vi "GOOP_AddCustomClassTemplates.vi"(7 "DerivedFromThisClass(if any)":refnum<vi>, 9 "BuildInTemplates":string[](array[string]), 10 "TemplateIdNamesIn":T2[](array[typedef]), 11 "ClassWriter in":refnum<class "ClassWriter.lvclass">) -> (2 "TemplateIdNamesOut":T2[](array[typedef]))   [LabVIEW 2020]
uses:
  <resource>/Framework/Providers/Open_GDS/ClassProviders/Provider_BaseClassInterface/ClassTemplateType.ctl
  <resource>/Framework/Providers/Open_GDS/ClassProviders/Provider_BaseClassInterface/ClassWriter_class/ClassWriter.lvclass
  <resource>/Framework/Providers/Open_GDS/ClassProviders/Common/ScriptingFunctions/Scripting_ConnectorPanePatternType.ctl
panel:
  out "PatternOut":T1 items=["4x4x4", "5x6x5", "6x8x6"]
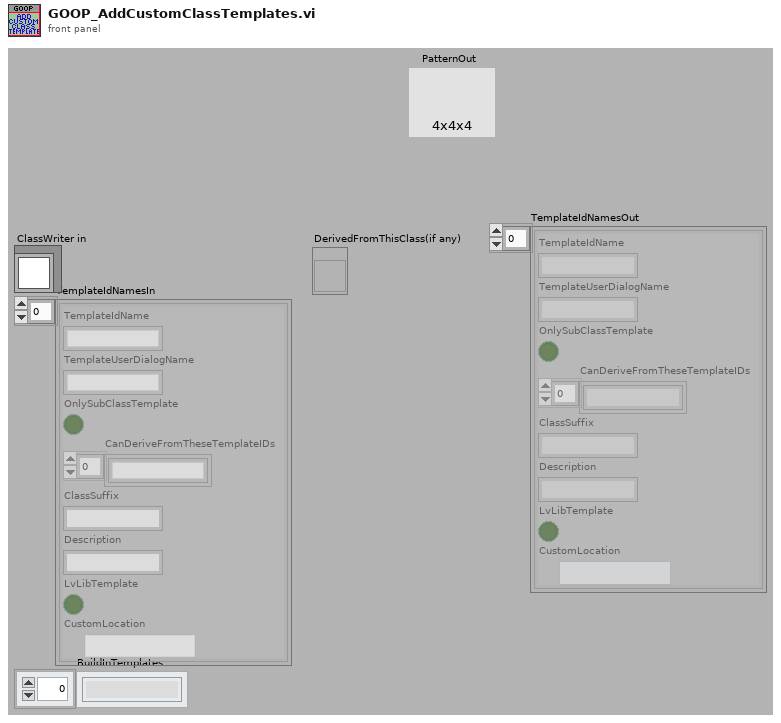
[diagram p1: front panel]
types:
  T1 = typedef "Scripting_ConnectorPanePatternType.ctl" = u16
  T2 = typedef "ClassWriter.lvclass/ClassTemplateType.ctl" = cluster{"TemplateIdName":string, "TemplateUserDialogName":string, "OnlySubClassTemplate":bool, "CanDeriveFromTheseTemplateIDs":string[], "ClassSuffix":string, "Description":string, "LvLibTemplate":bool, "CustomLocation":path}
  T3 = typedef "GDSLvCLass_ClassSettingsType.ctl" = cluster{"ClassProviderName":string, "ClassTemplateUsed":string, "ClassTemplateVersion":string, "ClassDescription":string, "PlugIns":T4[], "ConnectorPanePattern":string}
  T4 = typedef "GDSLvClass_PlugIn.ctl" = cluster{"Type":T5, "ID":string, "Version":string, "Path":path, "Name":string, "Data":variant}
  T5 = typedef "GDSLvClass_PlugInTypes.ctl" = enum16{"DesignPattern", "MethodTypes"}
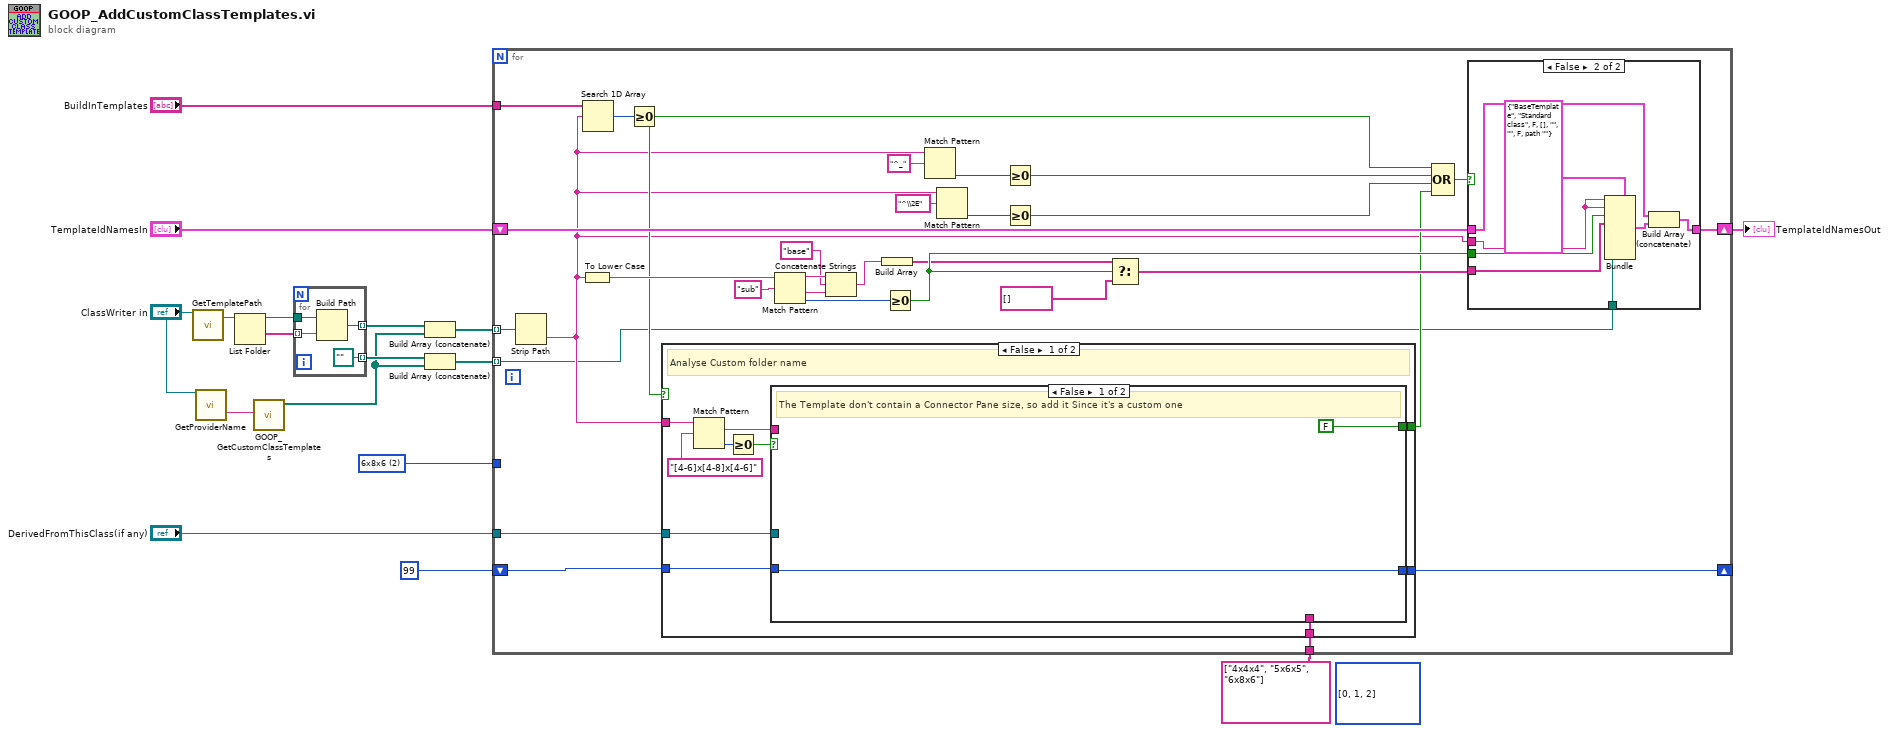
[diagram p0: block diagram]
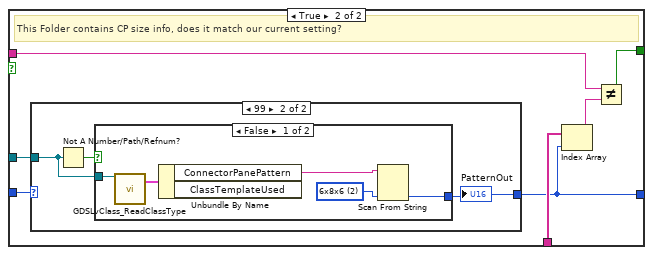
[diagram p2: hidden frame]
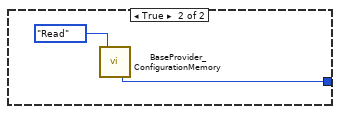
[diagram p4: hidden frame]
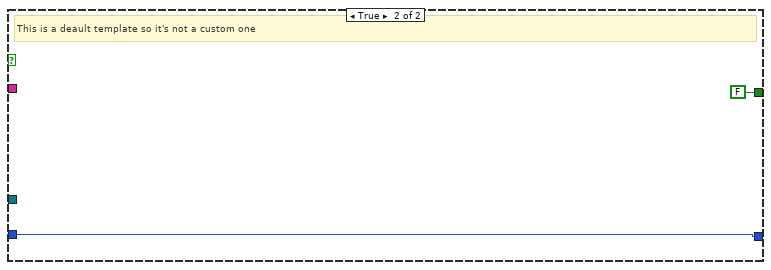
[diagram p5: hidden frame]
diagram:
  w11 = T1 2 items=["4x4x4", "5x6x5", "6x8x6"] ("_DefaultConnectorPanePattern")
  (unwired) T1[] [0, 1, 2] items=["4x4x4", "5x6x5", "6x8x6"] ("Pattern")
  n1 = call-dynamic "GetTemplatePath.vi"("ClassWriterIn"="ClassWriter in") -> ("FolderPathOut"=w15:path)  [unwired: 14 in, 4 out]
  n2 = call-dynamic "GetProviderName.vi"("ClassWriter in"="ClassWriter in") -> ("ShortName(Could be used in for INI Sections)"=w6:string)  [unwired: 14 in, 4 out]
  n3 = List Folder(path=w15) -> (path out=w8:path, folder names=w13:string[])  [unwired: 3 in, 2 out]
  n4 = call <resource>:"GOOP_GetCustomClassTemplates.vi"("ClassType"=w6) -> ("CustomTemplates"=w2:path[])  [unwired: 10 in]
  n5 = for {
    tunnel: w13 -> [w21] mode=indexing
    tunnel: w8 -> [w20]
    tunnel: [w19] -> w4 mode=indexing
    tunnel: [path ""] -> w3 mode=indexing
    n6 = Build Path(base path=w20, name or relative path=w21) -> (appended path=w19:path)
  }
  n7 = Build Array (concatenate)(w4, w2) -> (w5:path[])
  n8 = Build Array (concatenate)(w3, w2) -> (w1:path[])
  n9 = for {
    tunnel: "BuildInTemplates" -> [w32]
    shift-right: [w42] -> w16
    shift-left: "TemplateIdNamesIn" -> [w43]
    shift-right: [w28] -> _
    shift-left: u16 99 -> [w30]
    tunnel: w11 -> [_]
    tunnel: "DerivedFromThisClass(if any)" -> [w29]
    tunnel: string[] ["4x4x4", "5x6x5", "6x8x6"] ("Pattern") -> [w25]
    tunnel: w5 -> [w24] mode=indexing
    tunnel: w1 -> [w22] mode=indexing
    n10 = Strip Path(path=w24) -> (name=w23:string)  [unwired: 1 out]
    n11 = To Lower Case(string=w23) -> (all lower case string=w31:string)
    n12 = Search 1D Array(1D array=w32, element=w23) -> (index of element=w33:i32)  [unwired: 1 in]
    n13 = Greater Or Equal To 0?(x=w33) -> (x >= 0?=w26:bool)
    n14 = case shown="False" w26 {
      tunnel: w23 -> [w62 _]
      tunnel: w30 -> [w58 w84]
      tunnel: w29 -> [w57 _]
      tunnel: [w56 w84] -> w28
      tunnel: [w55 FALSE] -> w27
      tunnel: w25 -> [w54 _]
      frame False {
        # "Analyse Custom folder name"
        n15 = Match Pattern(string=w62, regular expression="[4-6]x[4-8]x[4-6]") -> (match substring=w53:string, offset past match=w60:i32)  [unwired: 1 in, 2 out]
        n16 = Greater Or Equal To 0?(x=w60) -> (x >= 0?=w59:bool)
        n17 = case shown="False" w59 {
          tunnel: w58 -> [w64 w71]
          tunnel: w57 -> [_ w70]
          tunnel: [w64 w68] -> w56
          tunnel: [FALSE w65] -> w55
          tunnel: w54 -> [_ w69]
          tunnel: w53 -> [_ w66]
          frame False {
            # "The Template don't contain a Connector Pane size, so add it Since it's a custom one"
          }
          frame True {
            # "This Folder contains CP size info, does it match our current setting?"
            n18 = case shown="99" w71 {
              selector: w71 -> [w72 _]
              tunnel: w70 -> [_ w74]
              tunnel: [w72 w73] -> w68
              frame 0, Default {
              }
              frame 99 {
                n19 = Not A Number/Path/Refnum?(number/path/refnum=w74) -> (NaN/Path/Refnum?=w75:bool)
                n20 = case shown="False" w75 {
                  tunnel: w74 -> [w77 _]
                  tunnel: [w76 w81] -> w73
                  frame False {
                    w78 = T1 2 items=["4x4x4", "5x6x5", "6x8x6"] ("Pattern")
                    n21 = call <resource>:"GDSLvClass_ReadClassType.vi"("Class Refnum In"=w77) -> ("ClassSettings"=w80:T3)  [unwired: 16 in, 2 out]
                    n22 = Unbundle By Name(w80) -> ("ConnectorPanePattern"=w79:string)  [unwired: 1 out]
                    n23 = Scan From String(input string=w79, default 1=w78) -> (output 1=w76:T1)  [unwired: 3 in, 3 out]
                  }
                  frame True {
                    n24 = call <resource>:"BaseProvider_ConfigurationMemory.vi"("Action"=enum16{"Read", "Load", "Save"}."Read") -> ("PatternOut"=w81:T1)  [unwired: 12 in, 6 out]
                  }
                }
                "PatternOut" <- w73
              }
            }
            n25 = Index Array(array=w69, index=w68) -> (element=w67:string)
            n26 = Not Equal?(x=w66, y=w67) -> (x != y?=w65:bool)
          }
        }
      }
      frame True {
        # "This is a deault template so it's not a custom one"
      }
    }
    n27 = Match Pattern(string=w31, regular expression="sub") -> (before substring=w41:string, after substring=w40:string, offset past match=w52:i32)  [unwired: 1 in, 1 out]
    n28 = Concatenate Strings(w41, "base" ("regular expression"), w40) -> (w37:string)
    n29 = Build Array(w37) -> (w36:string[])
    n30 = Greater Or Equal To 0?(x=w52) -> (x >= 0?=w38:bool)
    n31 = Match Pattern(string=w23, regular expression="^_") -> (offset past match=w44:i32)  [unwired: 1 in, 3 out]
    n32 = Match Pattern(string=w23, regular expression="^\\2E") -> (offset past match=w47:i32)  [unwired: 1 in, 3 out]
    n33 = Greater Or Equal To 0?(x=w44) -> (x >= 0?=w48:bool)
    n34 = Greater Or Equal To 0?(x=w47) -> (x >= 0?=w49:bool)
    n35 = Select(t=w36, s=w38, f=string[] []) -> (s? t:f=w35:string[])
    n36 = Compound Arithmetic op=OR(w26, w48, w49, w27) -> (w50:bool)
    n37 = case shown="False" w50 {
      tunnel: [w85 w93] -> w42
      tunnel: w43 -> [w85 w92]
      tunnel: w23 -> [_ w89]
      tunnel: w38 -> [_ w88]
      tunnel: w35 -> [_ w87]
      tunnel: w22 -> [_ w86]
      frame True {
        # "Don't add this template. It could be a default template or a custom that don't matches our CP"
      }
      frame False {
        n38 = Bundle(cluster=T2 {"TemplateIdName"="BaseTemplate", "TemplateUserDialogName"="Standard class", "OnlySubClassTemplate"=FALSE, "CanDeriveFromTheseTemplateIDs"=[], "ClassSuffix"="", "Description"="", "LvLibTemplate"=FALSE, "CustomLocation"=path ""} ("ClassTemplateType"), "TemplateIdName"=w89, "TemplateUserDialogName"=w89, "OnlySubClassTemplate"=w88, "CanDeriveFromTheseTemplateIDs"=w87, "CustomLocation"=w86) -> (w90:T2)  [unwired: 3 in]
        n39 = Build Array (concatenate)(w92, w90) -> (w93:T2[])
      }
    }
  }
  "TemplateIdNamesOut" <- w16
